vi "fake tool special labels.vi"(10 "Factor #1 & 50%":dbl, 11 "Length (mm)":dbl) -> (3 "Result (mm)":dbl)   [LabVIEW 2020, in "MCP Server tests.lvlib"]
doc: "This is a fake tool to test the MCP server toolkit. The labels of its inputs and of its output contain upper case letters, spaces, brackets and special characters, so their MCP names differ from the labels. It multiplies its two inputs, which are both required."
uses:
  MCP Server tests.lvlib
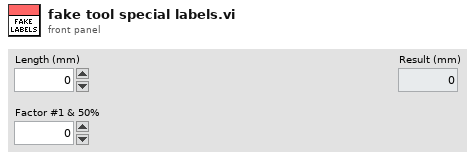
[diagram p1: front panel]
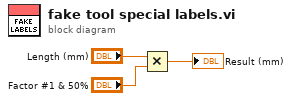
[diagram p0: block diagram]
diagram:
  n1 = Multiply(x="Length (mm)", y="Factor #1 & 50%") -> (x*y=→"Result (mm)":dbl)
